vi "measure BW6DB Measurement.vi"(8 "error in (no error)":errorcluster, 11 "SA Measurement in":refnum<class "SA Measurement.lvclass">) -> (0 "error out":errorcluster, 3 "SA Measurement out":refnum<class "SA Measurement.lvclass">)   [LabVIEW 2023, in "Spectrum Analyzer.lvlib" / "SA Measurement.lvclass"]
uses:
  SA Measurement.lvclass
  SA Measurement.lvclass/SA Measurement.ctl
  TYPE DEFINITION/Keysight 9020A/TYPE Measurement Preset.ctl
  Spectrum Analyzer.lvlib
  TYPE DEFINITION/TYPE RBW and VBW Select.ctl
  Interface_Spectrum/Interface_Spectrum.lvclass
  TYPE DEFINITION/TYPE Marker Peak Search Type.ctl
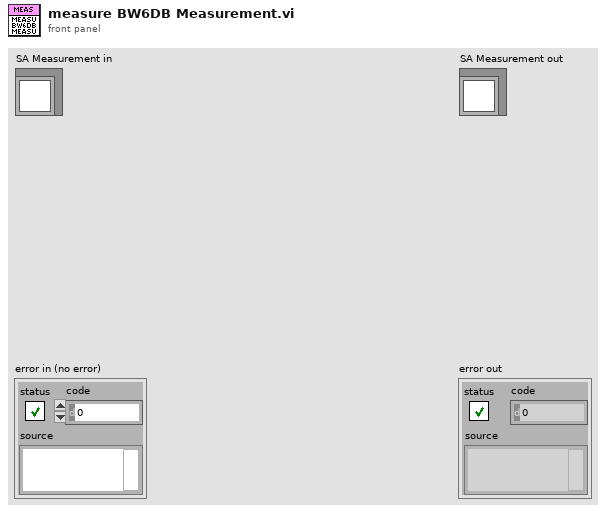
[diagram p1: front panel]
types:
  T1 = typedef "Spectrum Analyzer.lvlib/TYPE Marker Peak Search Type.ctl" = enum16{"Max", "Next Peak"}
  T2 = typedef "Spectrum Analyzer.lvlib/TYPE RBW and VBW Select.ctl" = enum16{"Res BW", "Video BW"}
  T3 = typedef "Spectrum Analyzer.lvlib/TYPE Measurement Preset.ctl" = enum16{"Sweep SA Mode", "Channel Power", "Occupied BW", "ACP", "Spurious Emission", "Spurious Emission Mask", "Burst Power (Transmit Power)"}
  T4 = typedef "Spectrum Analyzer.lvlib/TYPE Y-axis Unit.ctl" = enum16{"dBm", "dBmV", "dBuV", "dBpW", "Volt", "Ampere", "Watt"}
  T5 = typedef "Spectrum Analyzer.lvlib/TYPE Reference Level and Atten Param.ctl" = cluster{"Reference Level":dbl, "Atten":i32, "Atten Auto?":bool, "Reference Level Offset":dbl}
  T6 = typedef "Spectrum Analyzer.lvlib/TYPE Display Trace Mode Select.ctl" = enum16{"Clear Write", "Max Hold", "Min Hold", "Average", "View"}
  T7 = typedef "Spectrum Analyzer.lvlib/TYPE Detect Mode Select.ctl" = enum16{"Det Auto (Normal)", "Auto Peak", "Positive Peak", "Negative Peak", "Sample", "RMS", "Average", "Quasipeak", "CISPR Average", "RMS Average"}
  T8 = cluster{"Trace Mode":T6, "Detector Type":T7, "Detect Auto?":bool}[]
  T9 = typedef "Spectrum Analyzer.lvlib/TYPE OBW Measurement.ctl" = cluster{"Occupied BW (Hz)":dbl, "Total Power or OBW Power - dBm":dbl, "Transmit Frequency Error (Hz)":dbl, "x DB Bandwidth (Hz)":dbl, "Lower OBW Frequency (Hz)":dbl, "Upper OBW Frequency (Hz)":dbl}
  T10 = typedef "Spectrum Analyzer.lvlib/TYPE Marker Value.ctl" = cluster{"X-axis":dbl, "Y-axis":dbl}
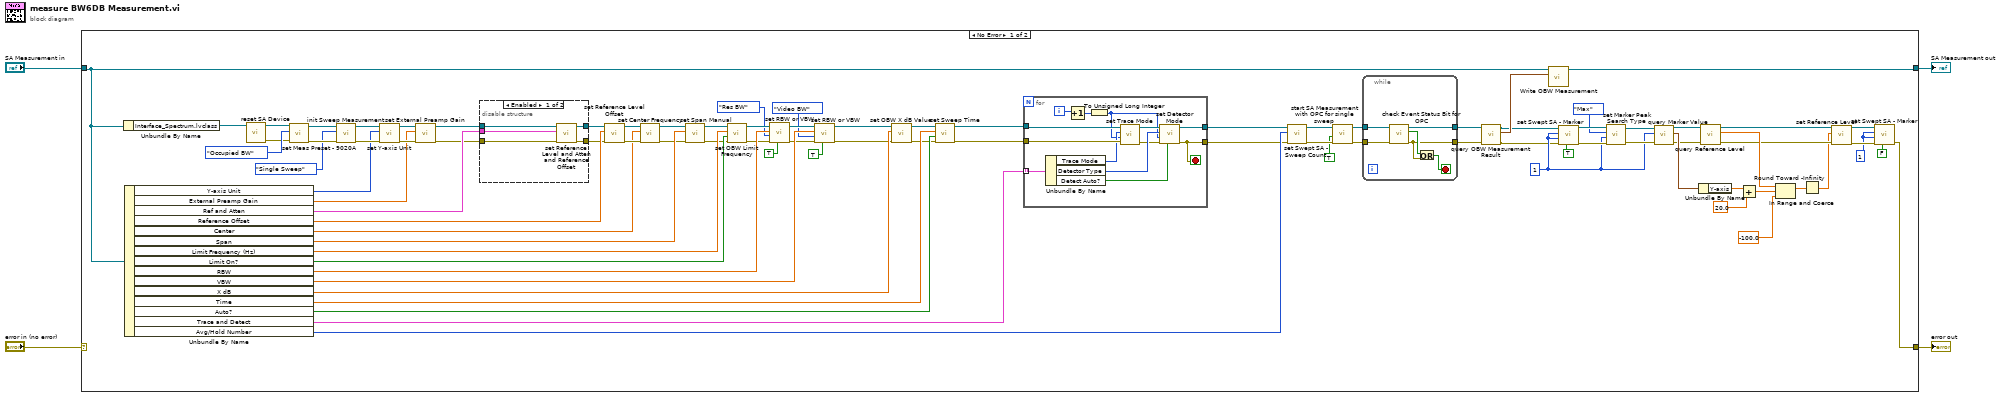
[diagram p0: block diagram]
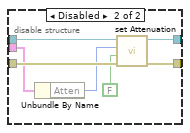
[diagram p2: hidden frame]
diagram:
  n1 = case shown="No Error" "error in (no error)" {
    selector: "error in (no error)" -> [_ w125]
    tunnel: [w5 w125] -> w3
    tunnel: [w31 w124] -> w1
    tunnel: "SA Measurement in" -> [w33 w124]
    frame No Error {
      w6 = 1 ("Index")
      w24 = 1 ("Index")
      n2 = Unbundle By Name(w33) -> ("Interface_Spectrum.lvclass"=w73:refnum<class "Interface_Spectrum.lvclass">)
      n3 = Unbundle By Name(w33) -> ("Y-axis Unit"=w81:T4, "External Preamp Gain"=w66:dbl, "Ref and Atten"=w88:T5, "Reference Offset"=w87:dbl, "Center"=w84:dbl, "Span"=w61:dbl, "Limit Frequency (Hz)"=w65:dbl, "Limit On?"=w64:bool, "RBW"=w56:dbl, "VBW"=w50:dbl, "X dB"=w63:dbl, "Time"=w44:dbl, "Auto?"=w43:bool, "Trace and Detect"=w80:T8, "Avg/Hold Number"=w79:u32)
      n4 = call-dynamic "reset SA Device.vi"("Interface_Spectrum in"=w73) -> ("error out"=w71:errorcluster, "Interface_Spectrum out"=w72:refnum<class "Interface_Spectrum.lvclass">)  [unwired: 9 in]
      n5 = call-dynamic "set Meas Preset - 9020A.vi"("error in (no error)"=w71, "Measurement Preset"=TYPE_Measurement_Preset."Occupied BW", "Interface_Spectrum in"=w72) -> ("error out"=w90:errorcluster, "Interface_Spectrum out"=w91:refnum<class "Interface_Spectrum.lvclass">)  [unwired: 7 in]
      n6 = call-dynamic "init Sweep Measurement.vi"("error in (no error)"=w90, "Sweep Measurement Mode"=enum16{"Single Sweep", "Continuous Sweep"}."Single Sweep", "Interface_Spectrum in"=w91) -> ("error out"=w82:errorcluster, "Interface_Spectrum out"=w83:refnum<class "Interface_Spectrum.lvclass">)  [unwired: 7 in]
      n7 = call-dynamic "set Y-axis Unit.vi"("error in (no error)"=w82, "Y-axis Unit"=w81, "Interface_Spectrum in"=w83) -> ("error out"=w69:errorcluster, "Interface_Spectrum out"=w70:refnum<class "Interface_Spectrum.lvclass">)  [unwired: 7 in]
      n8 = call-dynamic "set External Preamp Gain.vi"("error in (no error)"=w69, "External Preamp Gain (dB)"=w66, "Interface_Spectrum in"=w70) -> ("error out"=w67:errorcluster, "Interface_Spectrum out"=w68:refnum<class "Interface_Spectrum.lvclass">)  [unwired: 7 in]
      n9 = disable-structure shown="Enabled" {
        disable-tunnel: w88 -> [w97 w100]
        disable-tunnel: w68 -> [w96 w104]
        disable-tunnel: w67 -> [w95 w103]
        disable-tunnel: [w94 w102] -> w39
        disable-tunnel: [w93 w101] -> w38
        frame Enabled {
          n10 = call-dynamic "set Reference Level and Atten and Reference Offset.vi"("error in (no error)"=w95, "Reference Level, Atten, Reference Offset"=w97, "Interface_Spectrum in"=w96) -> ("error out"=w93:errorcluster, "Interface_Spectrum out"=w94:refnum<class "Interface_Spectrum.lvclass">)  [unwired: 7 in]
        }
        frame Disabled {
          n11 = Unbundle By Name(w100) -> ("Atten"=w99:i32)
          n12 = call-dynamic "set Attenuation.vi"("error in (no error)"=w103, "Auto?"=FALSE, "Attenuation"=w99, "Interface_Spectrum in"=w104) -> ("error out"=w101:errorcluster, "Interface_Spectrum out"=w102:refnum<class "Interface_Spectrum.lvclass">)  [unwired: 6 in]
        }
      }
      n13 = call-dynamic "set Reference Level Offset.vi"("error in (no error)"=w38, "Reference Level Offset"=w87, "Interface_Spectrum in"=w39) -> ("error out"=w85:errorcluster, "Interface_Spectrum out"=w86:refnum<class "Interface_Spectrum.lvclass">)  [unwired: 7 in]
      n14 = call-dynamic "set Center Frequency.vi"("error in (no error)"=w85, "Center Frequency (Hz)"=w84, "Interface_Spectrum in"=w86) -> ("error out"=w60:errorcluster, "Interface_Spectrum out"=w62:refnum<class "Interface_Spectrum.lvclass">)  [unwired: 7 in]
      n15 = call-dynamic "set Span Manual.vi"("error in (no error)"=w60, "Span (Hz)"=w61, "Interface_Spectrum in"=w62) -> ("error out"=w58:errorcluster, "Interface_Spectrum out"=w59:refnum<class "Interface_Spectrum.lvclass">)  [unwired: 7 in]
      n16 = call-dynamic "set OBW Limit Frequency.vi"("error in (no error)"=w58, "Limit On?"=w64, "Limit Frequency (Hz)"=w65, "Interface_Spectrum in"=w59) -> ("error out"=w54:errorcluster, "Interface_Spectrum out"=w57:refnum<class "Interface_Spectrum.lvclass">)  [unwired: 6 in]
      n17 = call-dynamic "set RBW or VBW.vi"("BW Auto?"=TRUE, "error in (no error)"=w54, "BW Type"=TYPE_RBW_and_VBW_Select."Res BW", "BW Value (Hz)"=w56, "Interface_Spectrum in"=w57) -> ("error out"=w48:errorcluster, "Interface_Spectrum out"=w51:refnum<class "Interface_Spectrum.lvclass">)  [unwired: 5 in]
      n18 = call-dynamic "set RBW or VBW.vi"("BW Auto?"=TRUE, "error in (no error)"=w48, "BW Type"=TYPE_RBW_and_VBW_Select."Video BW", "BW Value (Hz)"=w50, "Interface_Spectrum in"=w51) -> ("error out"=w46:errorcluster, "Interface_Spectrum out"=w47:refnum<class "Interface_Spectrum.lvclass">)  [unwired: 5 in]
      n19 = call-dynamic "set OBW X dB Value.vi"("error in (no error)"=w46, "OBW X dB (minus Value)"=w63, "Interface_Spectrum in"=w47) -> ("error out"=w42:errorcluster, "Interface_Spectrum out"=w45:refnum<class "Interface_Spectrum.lvclass">)  [unwired: 7 in]
      n20 = call-dynamic "set Sweep Time.vi"("error in (no error)"=w42, "Sweep Time Auto?"=w43, "Sweep Time(sec)"=w44, "Interface_Spectrum in"=w45) -> ("error out"=w40:errorcluster, "Interface_Spectrum out"=w41:refnum<class "Interface_Spectrum.lvclass">)  [unwired: 6 in]
      n21 = for {
        tunnel: w41 -> [w122]
        tunnel: w40 -> [w121]
        tunnel: w80 -> [w123] mode=indexing
        tunnel: [w111] -> w36
        tunnel: [w112] -> w37
        i -> [w120]
        stop <- w111 stop-if-true
        n22 = Unbundle By Name(w123) -> ("Trace Mode"=w118:T6, "Detector Type"=w116:T7, "Detect Auto?"=w113:bool)
        n23 = Increment(x=w120) -> (x+1=w119:i32)
        n24 = To Unsigned Long Integer(number=w119) -> (unsigned 32bit integer=w114:u32)
        n25 = call-dynamic "set Trace Mode.vi"("error in (no error)"=w121, "Trace Index"=w114, "Trace Mode"=w118, "Interface_Spectrum in"=w122) -> ("error out"=w115:errorcluster, "Interface_Spectrum out"=w117:refnum<class "Interface_Spectrum.lvclass">)  [unwired: 6 in]
        n26 = call-dynamic "set Detector Mode.vi"("Detect Auto?"=w113, "error in (no error)"=w115, "Trace Index"=w114, "Detector Type"=w116, "Interface_Spectrum in"=w117) -> ("error out"=w111:errorcluster, "Interface_Spectrum out"=w112:refnum<class "Interface_Spectrum.lvclass">)  [unwired: 5 in]
      }
      n27 = call-dynamic "set Swept SA - Sweep Count.vi"("error in (no error)"=w36, "Sweep Count"=w79, "Interface_Spectrum in"=w37) -> ("error out"=w77:errorcluster, "Interface_Spectrum out"=w78:refnum<class "Interface_Spectrum.lvclass">)  [unwired: 7 in]
      n28 = call-dynamic "start SA Measurement with OPC for single sweep.vi"("error in (no error)"=w77, "with OPC?"=TRUE, "Interface_Spectrum in"=w78) -> ("error out"=w74:errorcluster, "Interface_Spectrum out"=w75:refnum<class "Interface_Spectrum.lvclass">)  [unwired: 7 in]
      n29 = while {
        tunnel: w75 -> [w110]
        tunnel: w74 -> [w109]
        tunnel: [w106] -> w34
        tunnel: [w105] -> w35
        stop <- w107 stop-if-true
        n30 = call-dynamic "check Event Status Bit for OPC.vi"("error in (no error)"=w109, "Interface_Spectrum in"=w110) -> ("error out"=w106:errorcluster, "OPC Bit Changed?"=w108:bool, "Interface_Spectrum out"=w105:refnum<class "Interface_Spectrum.lvclass">)  [unwired: 7 in]
        n31 = Or(x=w108, y=w106) -> (x .or. y?=w107:bool)
      }
      n32 = call-dynamic "query OBW Measurement Result.vi"("error in (no error)"=w34, "Interface_Spectrum in"=w35) -> ("error out"=w10:errorcluster, "OBW Measurement"=w32:T9, "Interface_Spectrum out"=w11:refnum<class "Interface_Spectrum.lvclass">)  [unwired: 7 in]
      n33 = call "Write OBW Measurement.vi"("OBW Measurement"=w32, "SA Measurement in"=w33) -> ("SA Measurement out"=w31:refnum<class "SA Measurement.lvclass">)  [unwired: 8 in, 1 out]
      n34 = call-dynamic "set Swept SA - Marker.vi"("On?"=TRUE, "error in (no error)"=w10, "trace"=w24, "Index"=w24, "Interface_Spectrum in"=w11) -> ("error out"=w28:errorcluster, "Interface_Spectrum out"=w29:refnum<class "Interface_Spectrum.lvclass">)  [unwired: 5 in]
      n35 = call-dynamic "set Marker Peak Search Type.vi"("error in (no error)"=w28, "Marker Index"=w24, "Peak Search Type"=TYPE_Marker_Peak_Search_Type."Max", "Interface_Spectrum in"=w29) -> ("error out"=w25:errorcluster, "Interface_Spectrum out"=w26:refnum<class "Interface_Spectrum.lvclass">)  [unwired: 6 in]
      n36 = call-dynamic "query Marker Value.vi"("error in (no error)"=w25, "Marker Index"=w24, "Interface_Spectrum in"=w26) -> ("error out"=w19:errorcluster, "Marker Value"=w21:T10, "Interface_Spectrum out"=w20:refnum<class "Interface_Spectrum.lvclass">)  [unwired: 6 in]
      n37 = Unbundle By Name(w21) -> ("Y-axis"=w23:dbl)
      n38 = call-dynamic "query Reference Level.vi"("error in (no error)"=w19, "Interface_Spectrum in"=w20) -> ("error out"=w14:errorcluster, "Ref Level"=w17:dbl, "Interface_Spectrum out"=w18:refnum<class "Interface_Spectrum.lvclass">)  [unwired: 7 in]
      n39 = Add(x=w23, y=20.0) -> (x+y=w16:dbl)
      n40 = In Range and Coerce(upper limit=w17, x=w16, lower limit=-100.0) -> (coerced(x)=w13:dbl)  [unwired: 1 out]
      n41 = Round Toward -Infinity(1:w13) -> (0:w12:dbl)
      n42 = call-dynamic "set Reference Level.vi"("error in (no error)"=w14, "Reference Level"=w12, "Interface_Spectrum in"=w18) -> ("error out"=w8:errorcluster, "Interface_Spectrum out"=w9:refnum<class "Interface_Spectrum.lvclass">)  [unwired: 7 in]
      n43 = call-dynamic "set Swept SA - Marker.vi"("On?"=FALSE, "error in (no error)"=w8, "trace"=w6, "Index"=w6, "Interface_Spectrum in"=w9) -> ("error out"=w5:errorcluster)  [unwired: 5 in, 1 out]
    }
    frame Error {
    }
  }
  "error out" <- w3
  "SA Measurement out" <- w1
